vi "Regresja_liniowa.vi"() -> ()   [LabVIEW 2026]
uses:
  <vilib>/Analysis/NI_AALPro.lvlib
panel:
  out "Regresja liniowa":cluster{"X":dbl[], "Best Linear Fit":dbl[]}[](graph)
  out "b":dbl
  out "a":dbl
  in  "Y":dbl[](array[numeric])
  in  "X":dbl[](array[numeric])
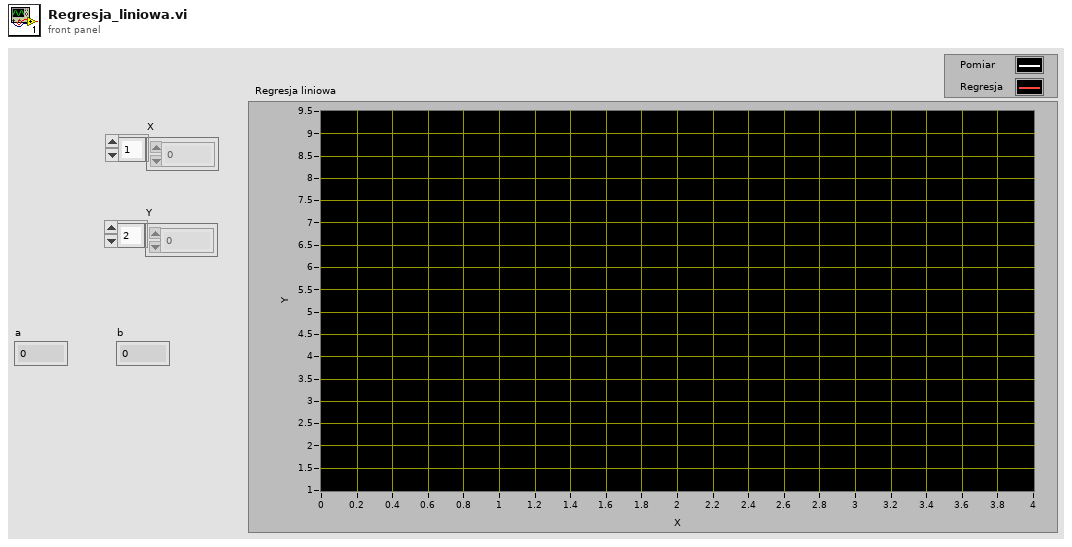
[diagram p1: front panel]
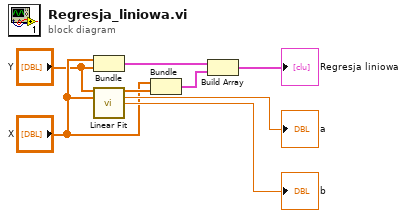
[diagram p0: block diagram]
diagram:
  n1 = Bundle("X"="X", "Y"="Y") -> (w1:cluster{"X":dbl[], "Y":dbl[]})  [unwired: 1 in]
  n2 = call <vilib>:"Linear Fit.vi"("Y"="Y", "X"="X") -> ("Best Linear Fit"=w6:dbl[], "slope"=→"a":dbl, "intercept"=→"b":dbl)  [unwired: 9 in, 2 out]
  n3 = Bundle("X"="X", "Best Linear Fit"=w6) -> (w5:cluster{"X":dbl[], "Best Linear Fit":dbl[]})  [unwired: 1 in]
  n4 = Build Array(w1, w5) -> (→"Regresja liniowa":cluster{"X":dbl[], "Best Linear Fit":dbl[]}[])
